vi "压力测量 - PS1.vi"(7 "CSM Name":string="PS1") -> ()   [LabVIEW 2026, in "UI-压力.lvlib"]
doc: "本范例执行串口读写操作。串口设置的参数必须匹配连接仪器或设备的参数。“VISA配置串口”VI可设置配置参数。前面板显示的控件可用于配置基本参数，如波特率、数据位和校验。VI会将VISA资源名称传递至其他VI以便执行相关操作。“VISA写入”函数将发送一个命令至串行设备，“VISA读取”函数将返回基于该命令的数据。“VISA关闭”函数可关闭该串行设备的引用。关闭引用十分重要，否则可能导致无法通过该端口进行进一步通信。"
uses:
  Supports/Device Info.ctl
  Data ColndSave/Supports/Time and Data.ctl
  <userlib>/_NEVSTOP/Communicable State Machine(CSM)/_Polymophic/CSM - Filter Duplicated Lines.vi
  3bfe9962-92bc-40b7-b1cd-a3f228b2ce0e.vi
  a504483a-bf88-4c5a-91ab-55111343aa78.vi
  83b94e39-b988-42ca-a5a6-ff8d58f134e6.vi
  5c51d1aa-81ea-4676-ad38-3af52935de4b.vi
  c16b87e5-7dba-47c4-ba33-901f1143b7c9.vi
  <userlib>/_NEVSTOP/Communicable State Machine(CSM)/_Polymophic/CSM - Replace Marks in Messages.vi
  3c314e7f-670f-419a-b1ed-a8d2dbf1e4a0.vi
  3d643602-a75e-4059-973b-e34c822a4a8c.vi
  373a0183-da7f-49bb-adc3-be145d208bff.vi
  943d190c-034f-4b86-a001-ad39c7e32d55.vi
  <userlib>/_NEVSTOP/Communicable State Machine(CSM)/AdvanceAPI/CSM - Compact Multiple States.vi
  <userlib>/_NEVSTOP/Communicable State Machine(CSM)/AdvanceAPI/CSM - Break Down Multiple States String.vi
  <userlib>/_NEVSTOP/Communicable State Machine(CSM)/_Shared/Remove Comments from Single-line.vi
  <userlib>/_NEVSTOP/Communicable State Machine(CSM)/_Shared/Split Single-line Message.vi
  <userlib>/_NEVSTOP/Communicable State Machine(CSM)/_Shared/Trim Single-line Text.vi
  <userlib>/_NEVSTOP/Communicable State Machine(CSM)/AdvanceAPI/CSM - Revert Arguments-Safe String.vi
  <userlib>/_NEVSTOP/Communicable State Machine(CSM)/AdvanceAPI/CSM - Make String Arguments Safe.vi
  5c51d1aa-81ea-4676-ad38-3af52935de4b.vi/99de0c97-112a-4c86-9094-c187659127e1.vi
  <userlib>/_NEVSTOP/Communicable State Machine(CSM)/Utility/Build Error Cluster.vi
  <vilib>/Utility/error.llb/Trim Whitespace.vi
  <vilib>/Utility/error.llb/Trim Whitespace (string).vi
  <userlib>/_NEVSTOP/Communicable State Machine(CSM)/AdvanceAPI/CSM - Keywords.vi
  <vilib>/Utility/error.llb/Trim Whitespace One-Sided.vi
  <userlib>/_NEVSTOP/Communicable State Machine(CSM)/addons/API-String-Arugments-Support/_Support/Data To API String Arguments.vi
  <userlib>/_NEVSTOP/Communicable State Machine(CSM)/addons/INI-Static-Variable-Support/_Support/instances/_CSM - Read File Logger Configuration - v1.0.vi
  <vilib>/Utility/Data Type/Get Type Information.vi
  <userlib>/_NEVSTOP/Communicable State Machine(CSM)/addons/API-String-Arugments-Support/_Support/Data To SingleElementsArray_csm.vi
  <userlib>/_NEVSTOP/Communicable State Machine(CSM)/addons/INI-Static-Variable-Support/_Support/Parse Used Session and Name.vi
  <userlib>/_NEVSTOP/Communicable State Machine(CSM)/addons/INI-Static-Variable-Support/_Support/INI-FGV(lvlibp).vi
  <userlib>/_NEVSTOP/Communicable State Machine(CSM)/addons/INI-Static-Variable-Support/_Support/Populate String with INI Variable.vi
  <userlib>/_NEVSTOP/Communicable State Machine(CSM)/addons/API-String-Arugments-Support/_Support/Convert API String Arguments to Data(variant).vi
  <userlib>/_NEVSTOP/Communicable State Machine(CSM)/addons/API-String-Arugments-Support/_Support/SingleElementsArray To Data_csm.vi
  <userlib>/_NEVSTOP/Communicable State Machine(CSM)/Communicable State Machine.lvlib
  <userlib>/_NEVSTOP/Communicable State Machine(CSM)/addons/INI-Static-Variable-Support/INI-Static-Variable-Support.lvlib
  <userlib>/_NEVSTOP/Communicable State Machine(CSM)/addons/MassData-Parameter/CSM MassData Parameter Support.lvlib
  <userlib>/_NEVSTOP/Communicable State Machine(CSM)/addons/Watchdog/CSM Watchdog.lvlib
  <userlib>/_NEVSTOP/Communicable State Machine(CSM)/addons/Logger/CSM File Logger.lvlib
  Logging/Logging.lvlib
  Acquisition/Acquisition.lvlib
  Data ColndSave/Data Collection and Save.lvlib
panel:
  in  "停止":bool
  in  "显示":enum32{"压力测量", "Status"}(tab)
  out "电压值":waveform(dbl)(graph)
  out "压力值(N)":dbl=0.5 format="%.3g"
  in  "压力设备选择":bool=TRUE
  in  "压力串口":refnum<visa-resource-name>="COM18"
  out "压力值(g)":dbl=0.5 format="%.3g"
  out "电压值":dbl=0.5 format="%.3g"
  in  "压力采集开关":bool
  out "压力(g)":waveform(dbl)(graph)
  in  "Interval(s)":dbl=0.5
  out "压力采集-错误输出":errorcluster
  out "State History":string
  in  "子程序？":bool
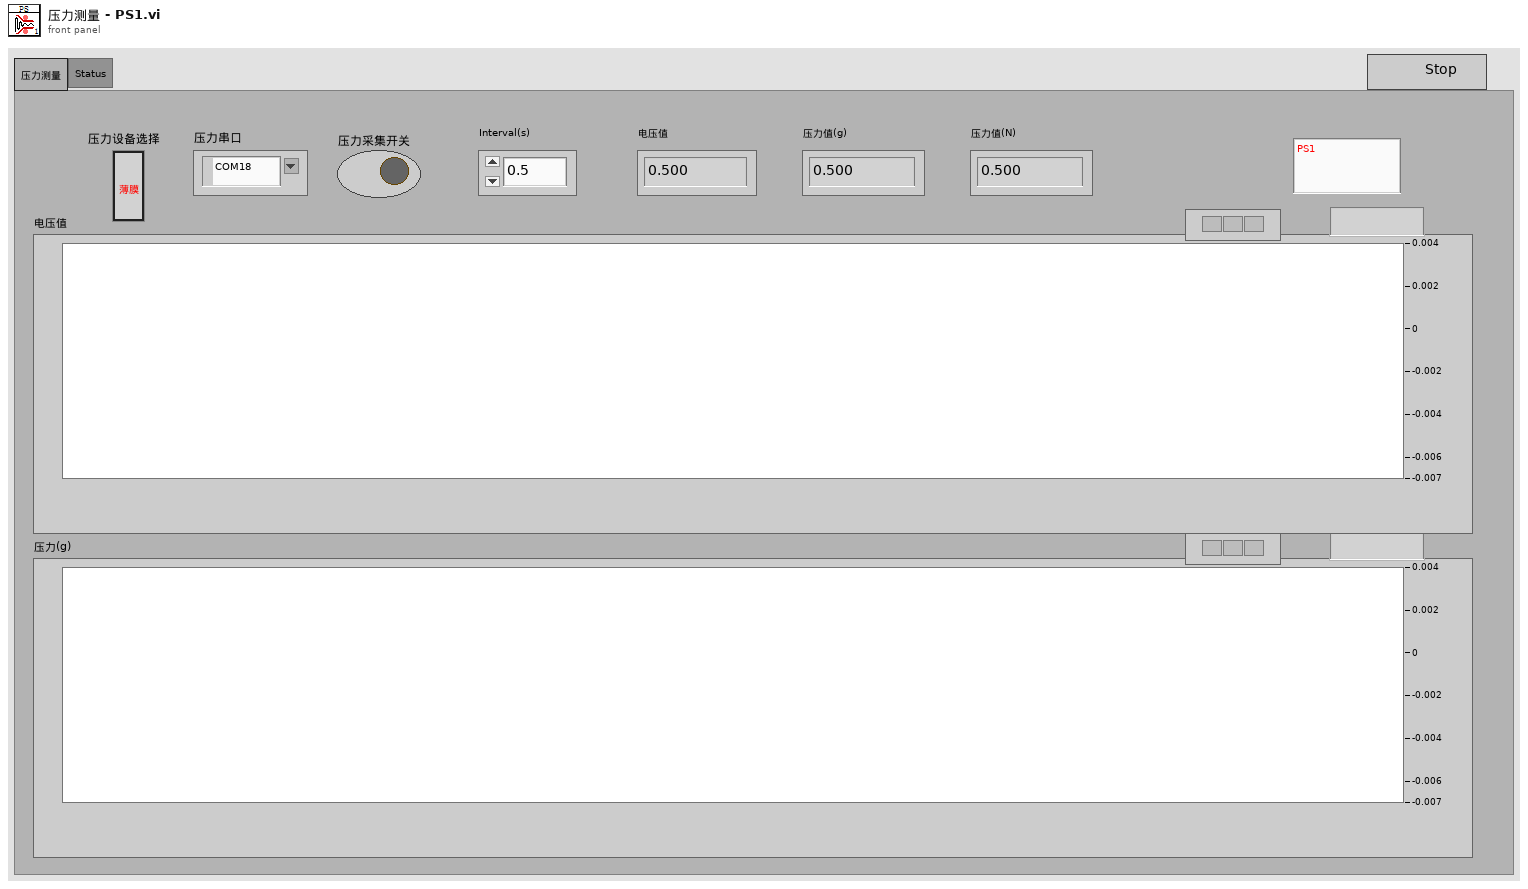
[diagram p1: front panel]
types:
  T1 = cluster{"Enable":bool, "Limit":cluster{"FileSize":i64, "FileNum":i32}, "Timestamp.Format":string, "AutoExit":bool}
  T2 = enum32{"Invalid", "Standard", "Closed", "Hidden", "Minimized", "Maximized"}
  T3 = enum32{"invalid app kind", "Development System", "Run Time System", "Student Edition", "Embedded LabVIEW", "Evaluation", "Custom"}
  T4 = typedef "Data Collection and Save.lvlib/Time and Data.ctl" = cluster{"采集时间":timestamp, "Data":dbl[]}
  T5 = typedef "Communicable State Machine.lvlib/_CSM_Response Source Message.ctl" = cluster{"‘State":string, "’Arguments":string, "’Error":errorcluster}
  T6 = cluster{"Current VI Reference":refnum<vi>, "Close Panel on Exit?":bool}
  T7 = typedef "UI-压力.lvlib/Device Info.ctl" = cluster{"USB Port":refnum<visa-resource-name>, "采集间隔(s)":dbl, "压力设备选择":bool}
  T8 = cluster{"Core":cluster{"Current VI Reference":refnum<vi>, "Close Panel on Exit?":bool}, "基本信息":T7, "Time and Data":T4, "子程序？":bool}
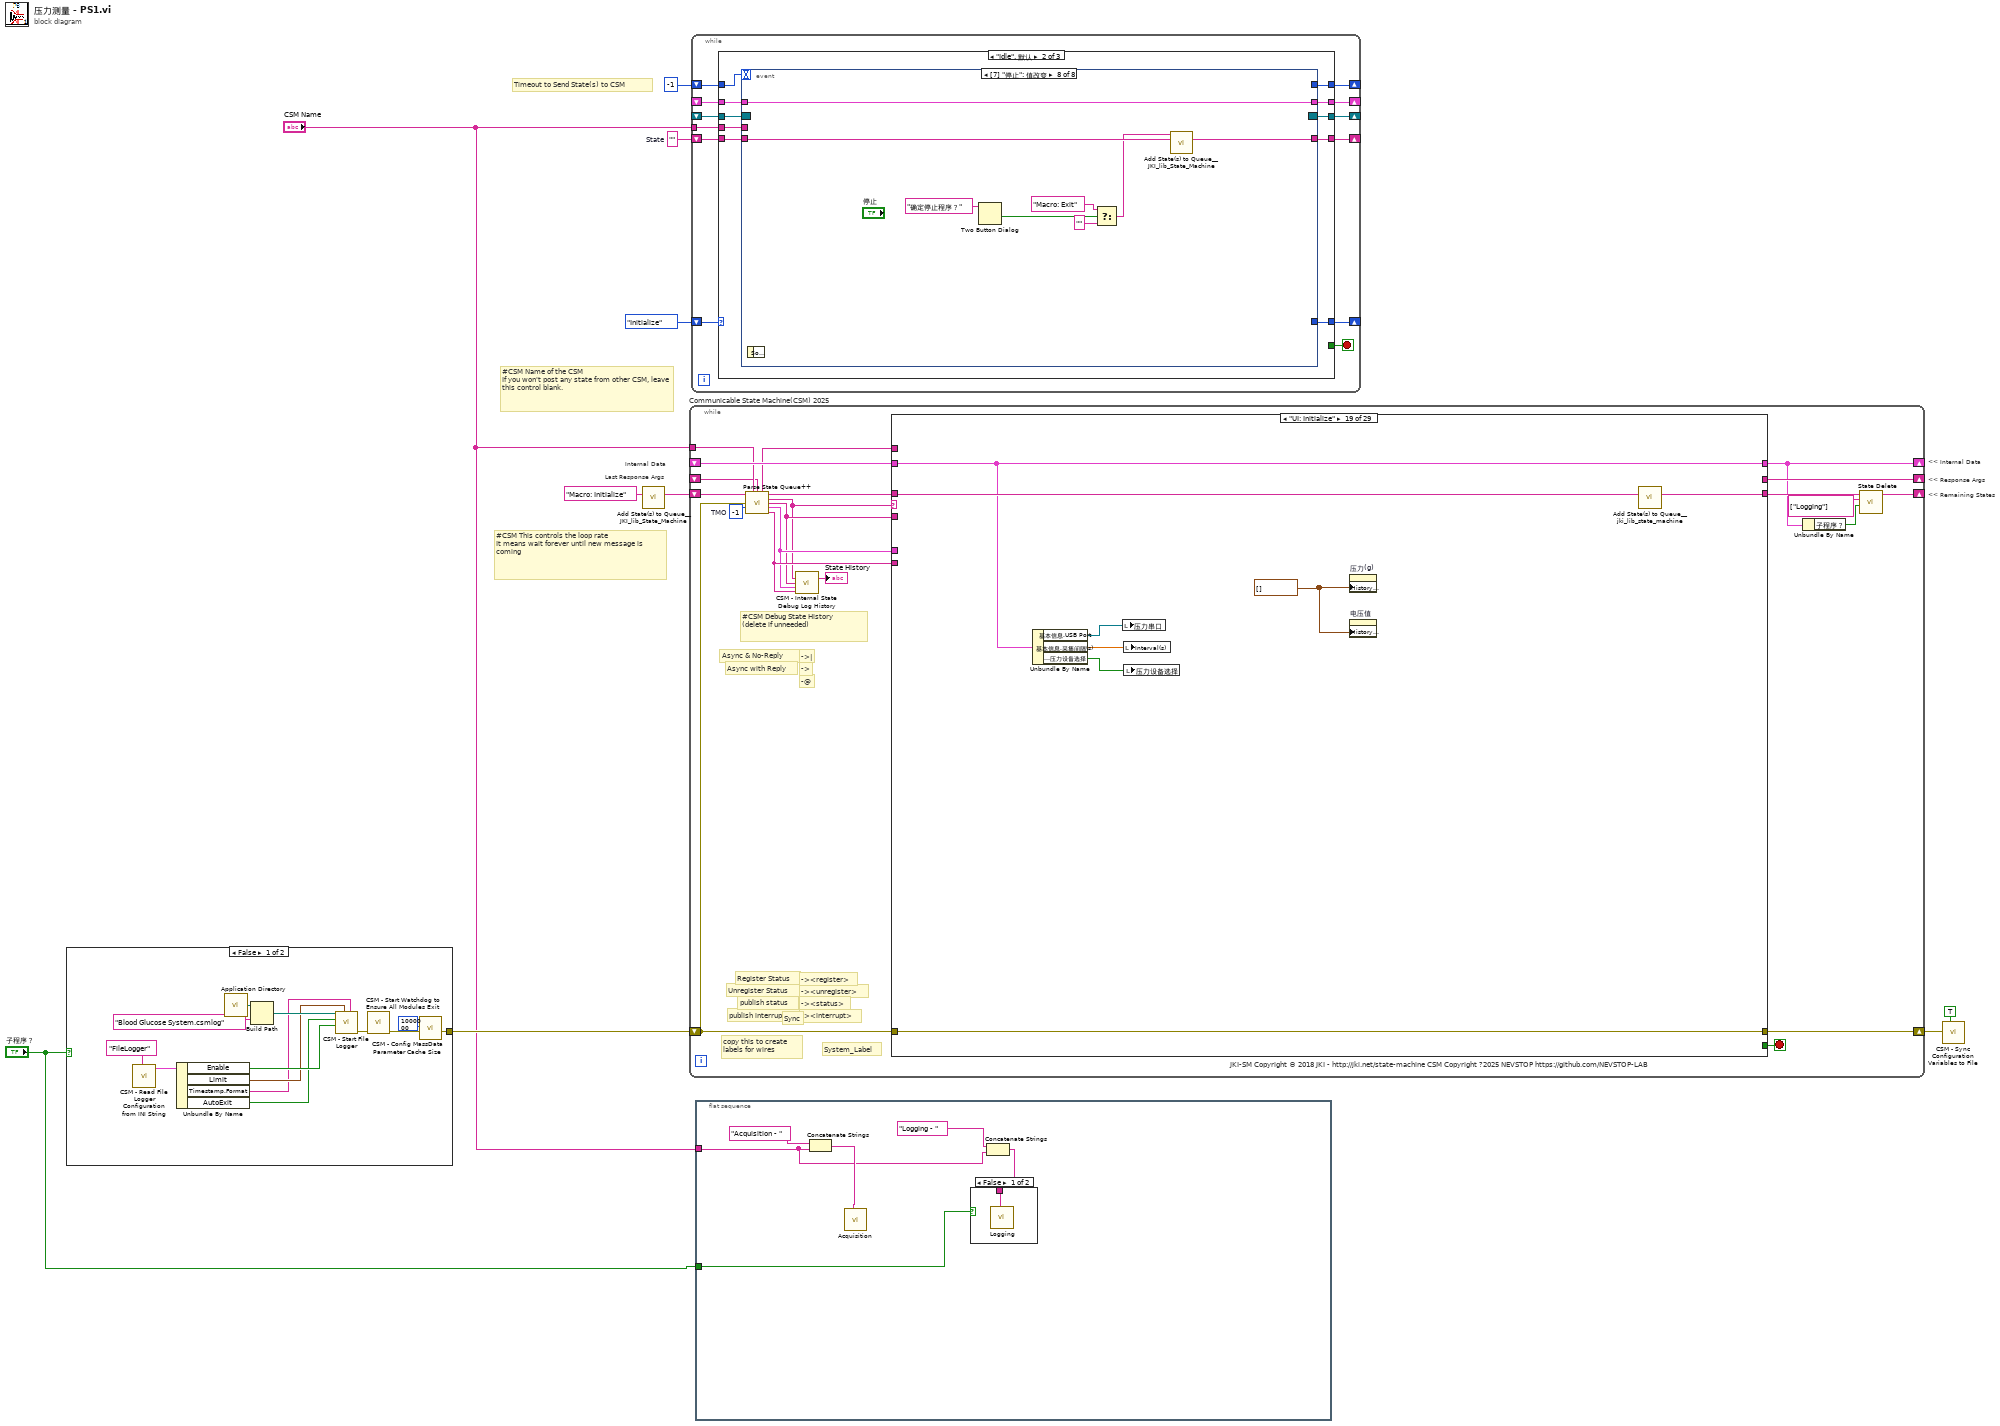
[diagram p0: block diagram]
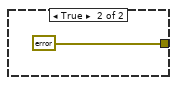
[diagram p3: hidden frame]
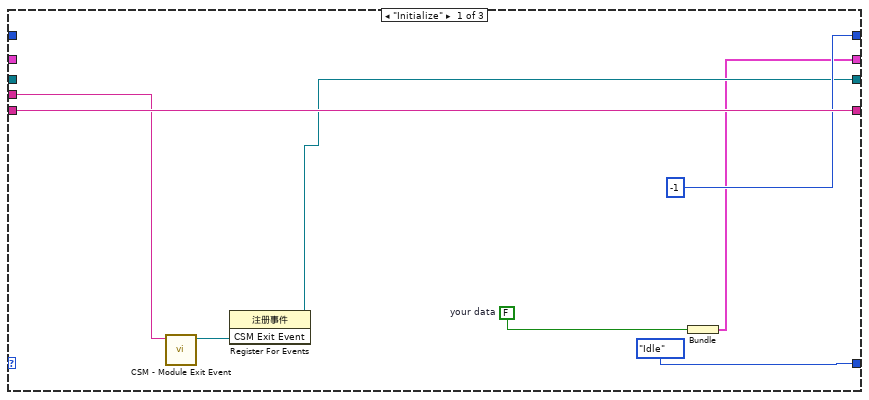
[diagram p4: hidden frame]
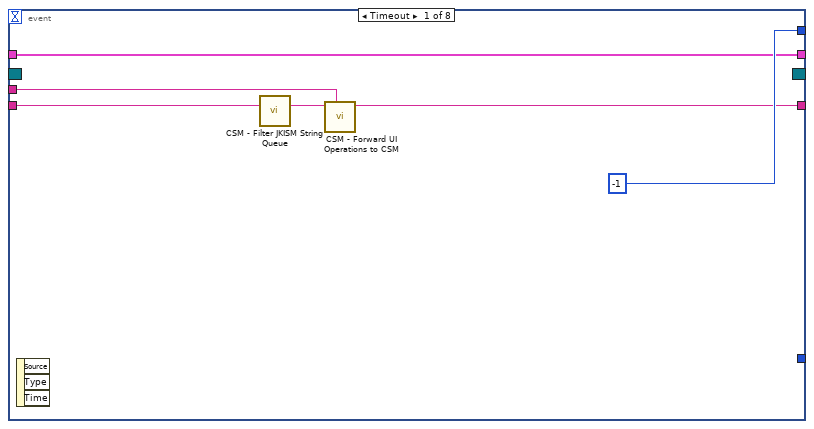
[diagram p5: hidden frame]
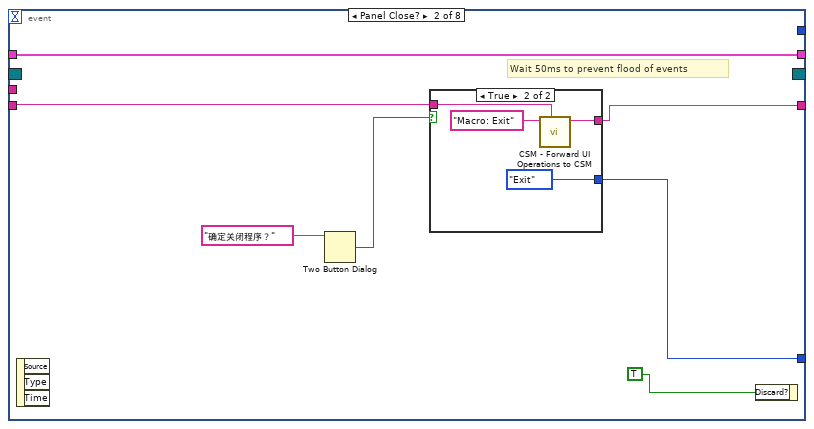
[diagram p6: hidden frame]
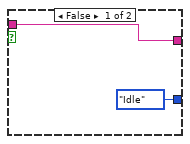
[diagram p7: hidden frame]
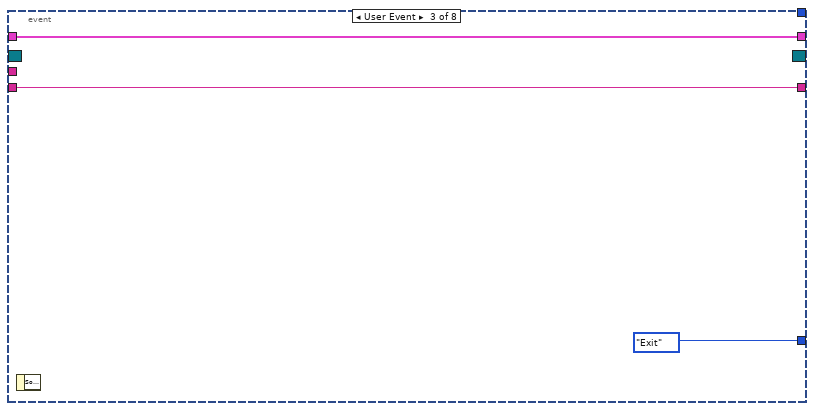
[diagram p8: hidden frame]
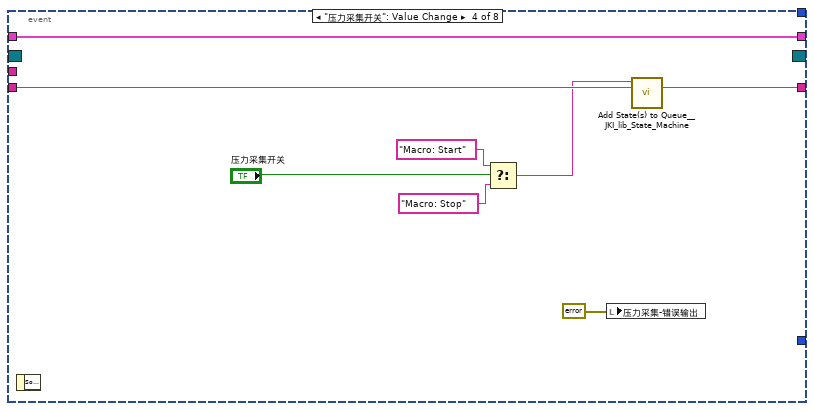
[diagram p9: hidden frame]
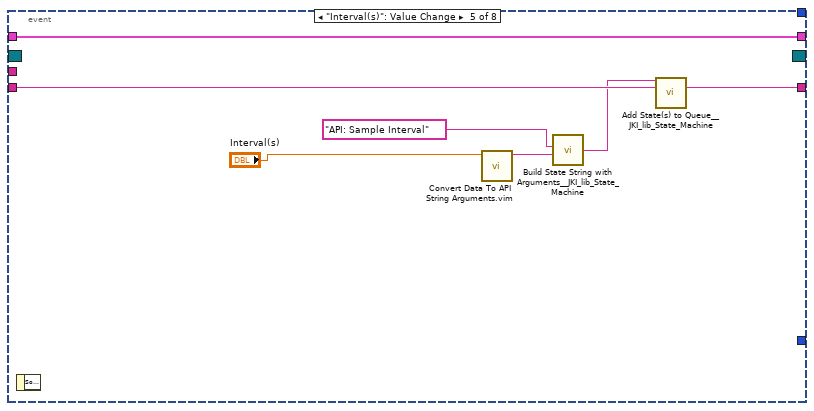
[diagram p10: hidden frame]
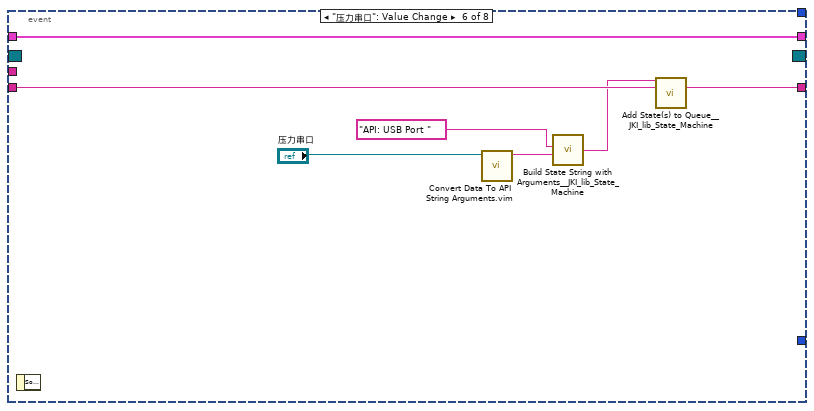
[diagram p11: hidden frame]
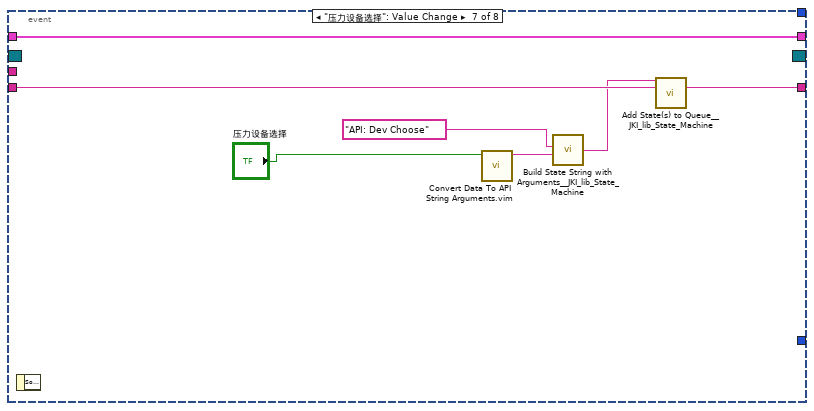
[diagram p12: hidden frame]
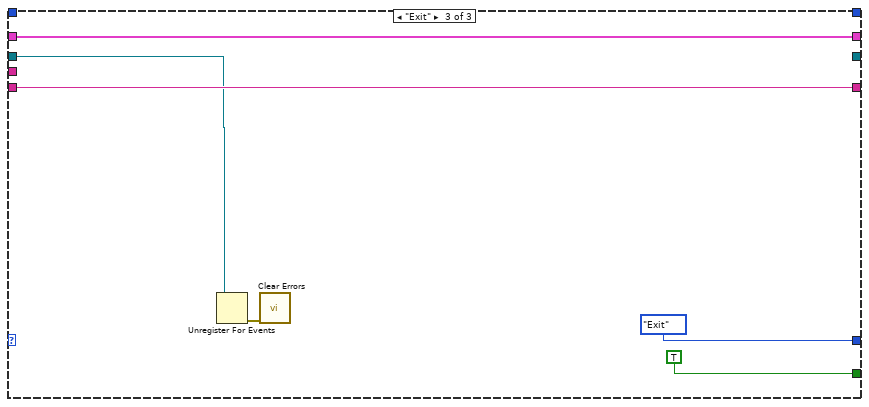
[diagram p13: hidden frame]
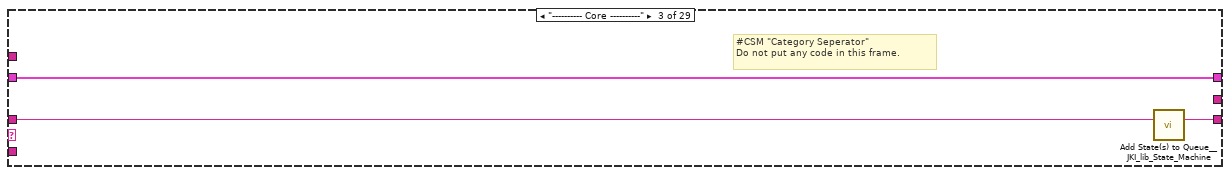
[diagram p16: hidden frame]
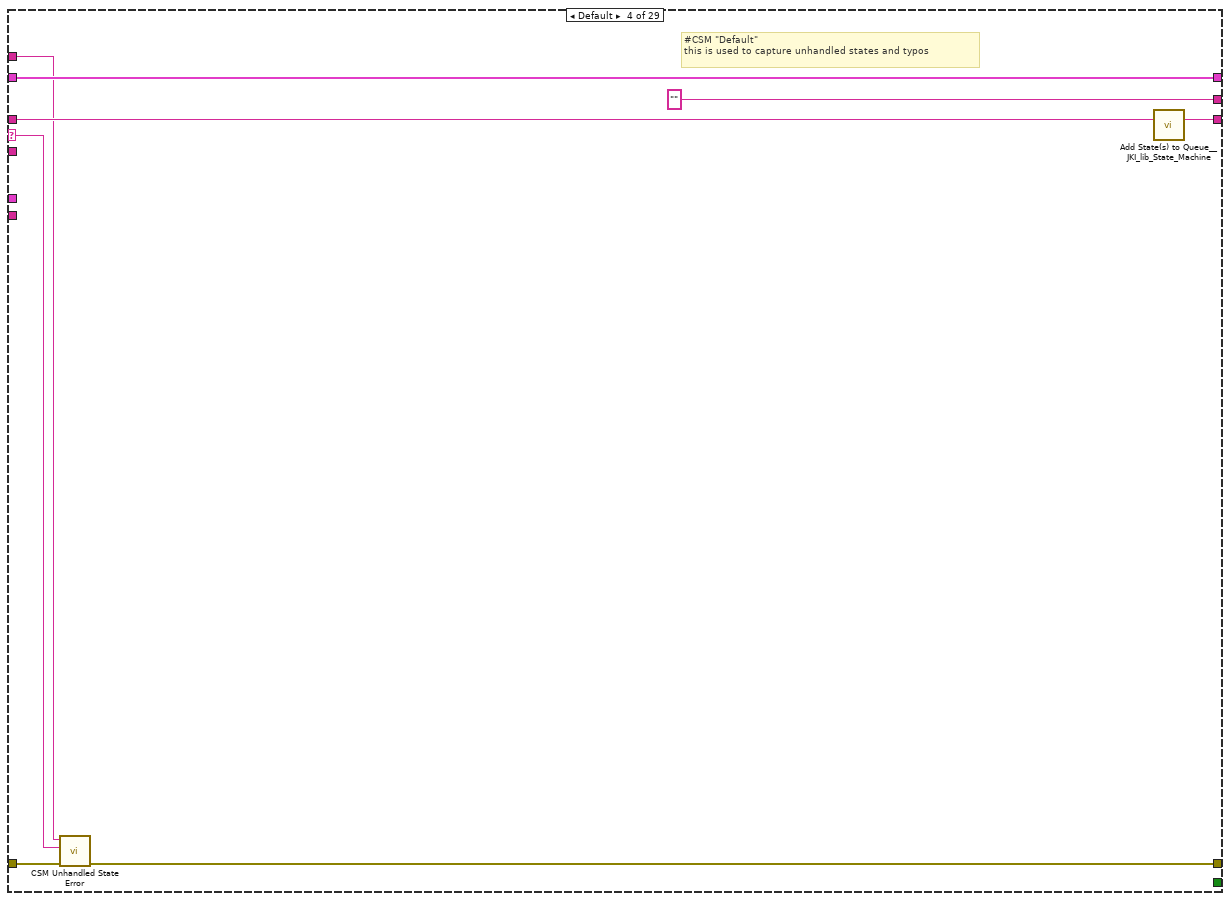
[diagram p17: hidden frame]
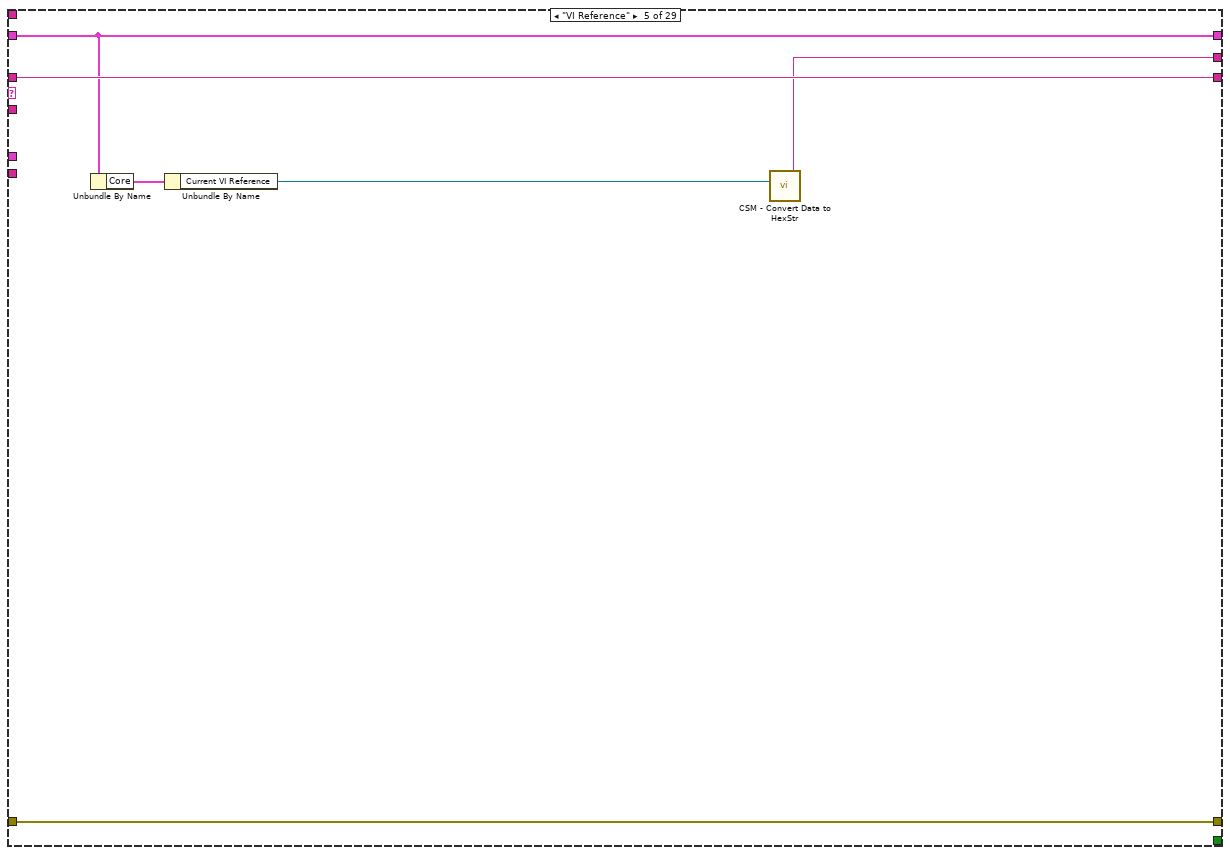
[diagram p18: hidden frame]
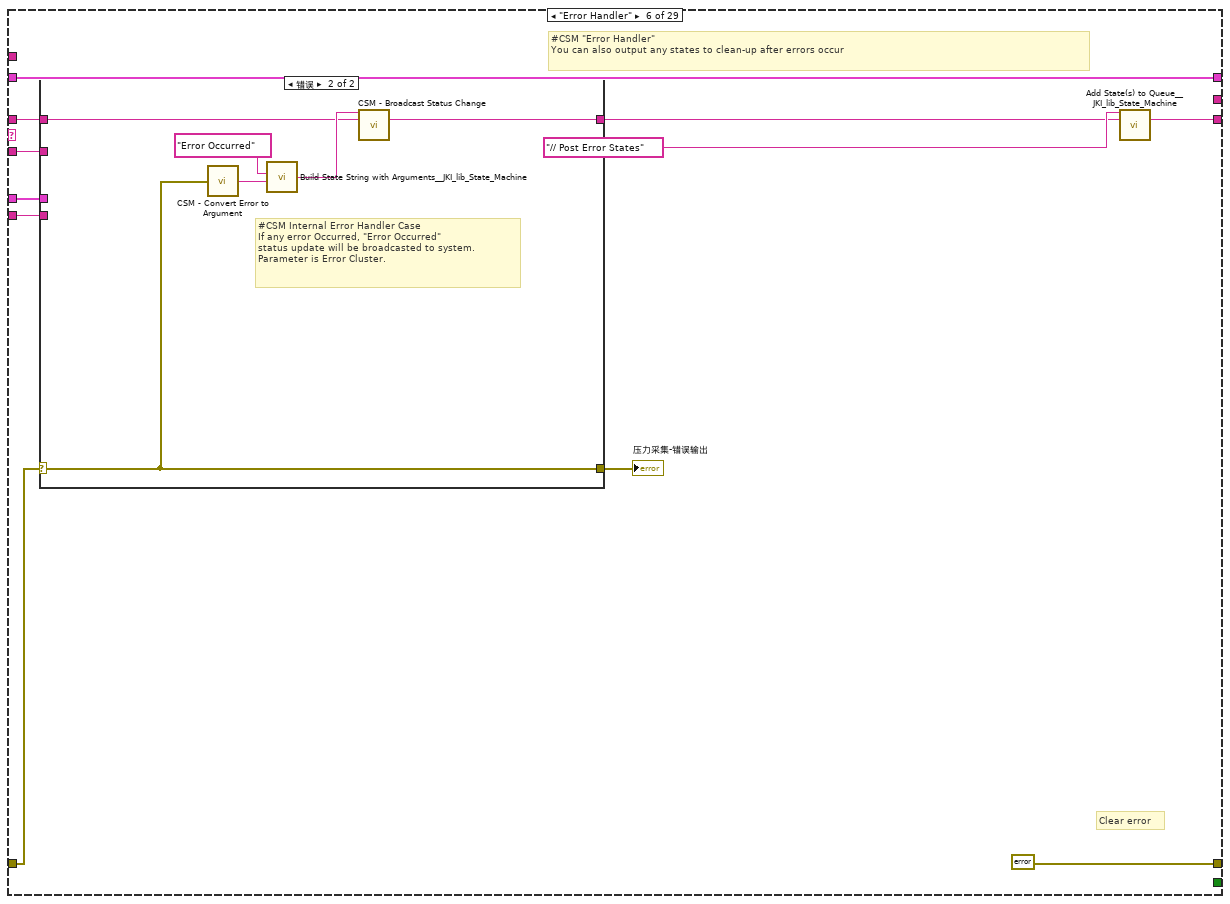
[diagram p19: hidden frame]
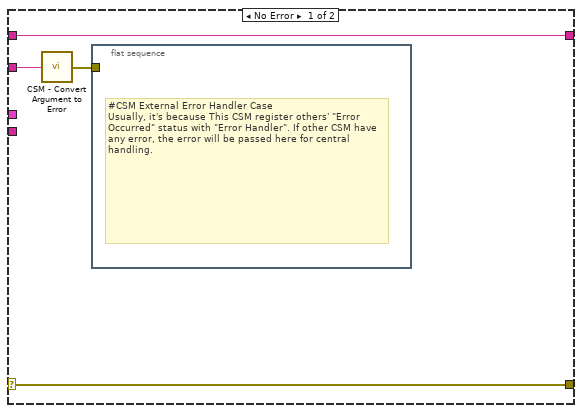
[diagram p20: hidden frame]
diagram:
  w9 = ""  # State
  # "Timeout to Send State(s) to CSM"
  # "Last Response Args"
  # "Internal Data"
  # "#CSM Name of the CSM\nIf you won't post any state from other CSM, leave this control blank."
  # "#CSM This controls the loop rate\nIt means wait forever until new message is coming"
  # "<< Internal Data"
  # "<< Response Args"
  # "<< Remaining States"
  n1 = case shown="False" "子程序？" {
    tunnel: [w21 errorcluster {"status"=FALSE, "code"=0, "source"=""} ("Error out")] -> w3
    frame False {
      n2 = call-poly <userlib>:"CSM - Read File Logger Configuration from INI String.vi"("Section Name(\"FileLogger\")"="FileLogger" ("Section Name(\"\" as Default)")) -> ("FileLogger Configuration-v1"=w15:T1)  [unwired: 7 in, 1 out]
      n3 = Unbundle By Name(w15) -> ("Enable"=w14:bool, "Limit"=w13:cluster{"FileSize":i64, "FileNum":i32}, "Timestamp.Format"=w11:string, "AutoExit"=w12:bool)
      n4 = call <vilib>:"Application Directory.vi"() -> ("Application Directory"=w20:path)
      n5 = Build Path(base path=w20, name or relative path="Blood Glucose System.csmlog") -> (appended path=w18:path)
      n6 = call <userlib>:"CSM - Start File Logger.vi"("Timestamp Format"=w11, "Log Limit"=w13, "Watchdog? (T)"=w14, "Exit When All Module Exist? (F)"=w12, "Log File Path"=w18) -> ("error out"=w17:errorcluster)  [unwired: 4 in, 2 out]
      n7 = call <userlib>:"CSM - Start Watchdog to Ensure All Modules Exit.vi"("error in (no error)"=w17) -> ("error out"=w22:errorcluster)  [unwired: 10 in]
      n8 = call <userlib>:"CSM - Config MassData Parameter Cache Size.vi"("Error in"=w22, "Size (50M)"=1000000 ("size(1M)")) -> ("Error out"=w21:errorcluster)  [unwired: 9 in]
    }
    frame True {
    }
  }
  n9 = call <vilib>:"Add State(s) to Queue__JKI_lib_State_Machine.vi"("State(s) in (\"\")"="Macro: Initialize" ("Init State(\"Macro: Initialize\")")) -> ("States Out"=w6:string)  [unwired: 14 in]
  n10 = while "Communicable State Machine(CSM) 2025" {
    shift-right: [w26] -> _
    shift-left: _ -> [w41]
    shift-right: [w43] -> w4
    shift-left: w3 -> [w31]
    shift-right: [w27] -> _
    shift-left: w6 -> [w44]
    tunnel: "CSM Name" -> [w38]
    shift-right: [w39] -> _
    shift-left: _ -> [w33]
    stop <- w42 stop-if-true
    w40 = -1  # TMO
    # "#CSM Debug State History\n(delete if unneeded)"
    # "-><interrupt>"
    # "-><status>"
    # "-><unregister>"
    # "-><register>"
    # "-@"
    # "->"
    # "->|"
    # "publish interrupt"
    # "publish status"
    # "Unregister Status"
    # "Register Status"
    # "Sync"
    # "Async with Reply"
    # "Async & No-Reply"
    # "JKI-SM Copyright © 2018 JKI - http://jki.net/state-machine CSM Copyright ?2025 NEVSTOP https://github.com/NEVSTOP-LAB"
    # "copy this to create labels for wires"
    # "System_Label"
    n11 = call <userlib>:"Parse State Queue++.vi"("State Queue"=w44, "Name (\"\" to Use UUID)"=w38, "Response Arguments"=w33, "Previous Error"=w31, "Dequeue (1 ms)"=w40) -> ("Name Used"=w32:string, "Remaining States"=w45:string, "Current State"=w34:string, "Arguments"=w35:string, "Additional Information"=w36:T5, "Source CSM"=w37:string)  [unwired: 5 in]
    n12 = call <userlib>:"CSM - Internal State Debug Log History.vi"("State"=w34, "Arguments (\"\")"=w35, ">> Response Source Message >>"=w36, "Source (\"\")"=w37) -> ("Debug Log"=→"State History":string)  [unwired: 11 in]
    n13 = case shown="\"UI: Initialize\"" w34 {
      selector: w34 -> [_ _ _ w56 _ _ _ _ _ _ _ _ _ _ _ _ _ _ _ _ _ _ _ _ _ _ _ _ _]
      tunnel: w45 -> [w46 w49 w52 w60 w65 w71 w95 w101 w107 w117 w124 w136 w140 w143 w156 w169 w178 w179 w188 w201 w206 w212 w221 w224 w235 w237 w245 w253 w260]
      tunnel: w35 -> [_ _ _ _ _ w70 w91 w98 w104 w111 _ _ _ _ _ w167 _ _ _ _ _ _ _ _ _ _ w242 w252 w259]
      tunnel: w41 -> [w47 w48 w50 w58 w64 w76 w93 w99 w105 w115 w123 w130 w138 w141 _ w160 w173 w181 w183 w193 w204 w210 w215 w228 w233 w236 w239 w250 w257]
      tunnel: [_ _ _ w53 w66 errorcluster {"status"=FALSE, "code"=0, "source"=""} ("error out") w88 w96 w102 w118 _ _ _ _ _ _ w174 w182 w190 w203 _ _ _ w229 _ _ _ _ _] -> w43
      tunnel: w31 -> [_ _ _ w54 w66 w74 w89 w97 w103 _ _ _ _ _ _ _ w175 w182 w190 w203 _ _ _ w229 _ _ _ _ _]
      tunnel: [w46 w49 w51 w59 w65 w72 w94 w100 w106 w116 w124 w135 w139 w142 w155 w170 w177 w180 w189 w202 w205 w211 w220 w225 w234 w237 w246 w254 w261] -> w28
      tunnel: [_ _ _ _ _ _ TRUE _ _ _ _ _ TRUE _ _ _ _ _ _ _ _ _ _ _ _ _ _ _ _] -> w42
      tunnel: [w47 w48 w50 w58 w64 w76 w93 w99 w105 w114 w123 w134 w138 w141 w154 w159 w173 w181 w183 w193 w204 w210 w216 w228 w233 w236 w238 w249 w256] -> w26
      tunnel: w37 -> [_ _ _ _ _ w69 _ _ _ w112 _ _ _ _ _ _ _ _ _ _ _ _ _ _ _ _ _ _ _]
      tunnel: w36 -> [_ _ _ _ _ w68 _ _ _ w113 _ _ _ _ _ _ _ _ _ _ _ _ _ _ _ _ _ _ _]
      tunnel: [_ _ _ "" w61 _ _ _ _ _ _ _ _ _ _ _ _ _ _ _ _ _ _ _ _ _ _ _ _] -> w39
      tunnel: w32 -> [_ _ _ w55 _ _ w90 _ _ _ _ _ _ _ w146 _ _ _ _ _ _ w208 _ w226 w230 _ w243 _ _]
      frame "", "Idle" {
        # "#CSM \"Idle/Event Handler\"\nexecutes when the state queue is empty"
      }
      frame "CSM Documentation" {
        # "#CSM State Syntax\n\n// Comment line, all text to the right of “//” will be ignored\n// Local Message Example\nDoSth: DoA >> Arguments\n\n// Sync Call Example\nAPI: xxxx >> Arguments -@ TargetModule\n\n// Async Call Example\nAPI: xxxx >> Arguments -> TargetModule\n\n// Async Call without Reply Example\nAPI: xxxx >> Arguments ->| TargetModule\n\n// Broadcast normal status:\nStatus >> StatusArguments  -><status>\n\n// Broadcast Interrupt status:\nInterrupt >> StatusArguments  -><interrupt>\n\n// Register Source Module's status to Handler Module\nStatus@Source Module >> Handler Module@Handler Module -><register>\n\n// Unegister Source Module's status\nStatus@Source Module >> Handler Module -><unregister>"
        # "#CSM README FIRST\n\nCommunicable State Machine(CSM) is a LabVIEW application framework that builds upon JKI State Machine(JKISM). It follows the pattern of JKISM and extends the keywords to describe message communication between modules, including concepts such as Sync-Message, Async-Message, Subscription/Unsubscription of status - essential elements for creating reusable code modules. For more information, please visit the CSM wiki: https://nevstop-lab.github.io/CSM-Wiki/\n\nFor instructions on JKI State Machine, visit: \n    http://jki.net/state-machine/\nFor information about CSM, visit: \n    https://github.com/NEVSTOP-LAB"
        # "#CSM \"Documentation\"\nCase for holding CSM Documenation"
      }
      frame "---------- Core ----------" {
        # "#CSM \"Category Seperator\"\nDo not put any code in this frame."
        n14 = call <vilib>:"Add State(s) to Queue__JKI_lib_State_Machine.vi"("State(s) in (\"\")"=w52) -> ("States Out"=w51:string)  [unwired: 14 in]
      }
      frame Default {
        # "#CSM \"Default\"\nthis is used to capture unhandled states and typos"
        n15 = call <userlib>:"CSM Unhandled State Error.vi"("error in (no error)"=w54, "Undefined State"=w56, "CSM Name"=w55) -> ("error out"=w53:errorcluster)  [unwired: 8 in]
        n16 = call <vilib>:"Add State(s) to Queue__JKI_lib_State_Machine.vi"("State(s) in (\"\")"=w60) -> ("States Out"=w59:string)  [unwired: 14 in]
      }
      frame "VI Reference" {
        n17 = Unbundle By Name(w64) -> ("Core"=w63:T6)
        n18 = Unbundle By Name(w63) -> ("Current VI Reference"=w62:refnum<vi>)
        n19 = call <userlib>:"CSM - Convert Data to HexStr.vi"("Variant"=w62) -> ("HEX String (0-9,A-F)"=w61:string)  [unwired: 8 in]
      }
      frame "Error Handler" {
        # "#CSM \"Error Handler\"\nYou can also output any states to clean-up after errors occur"
        # "Clear error"
        n20 = case shown="错误" w74 {
          selector: w74 -> [w78 w82]
          tunnel: [w81 w84] -> w73
          tunnel: w71 -> [w81 w83]
          tunnel: w70 -> [w80 _]
          tunnel: w69 -> [_ _]
          tunnel: w68 -> [_ _]
          tunnel: [w78 w82] -> w67
          frame No Error {
            n21 = call <userlib>:"CSM - Convert Argument to Error.vi"("Argument"=w80) -> ("Error"=w79:errorcluster)  [unwired: 4 in]
            n22 = flat-sequence {
              tunnel: w79 -> [_]
              frame #0 {
                # "#CSM External Error Handler Case\nUsually, it's because This CSM register others' \"Error Occurred\" status with \"Error Handler\". If other CSM have any error, the error will be passed here for central handling."
              }
            }
          }
          frame Error {
            # "#CSM Internal Error Handler Case \nIf any error Occurred, \"Error Occurred\" \nstatus update will be broadcasted to system.\nParameter is Error Cluster."
            n23 = call <userlib>:"CSM - Convert Error to Argument.vi"("Error"=w82) -> ("Argument"=w86:string)  [unwired: 4 in]
            n24 = call <vilib>:"Build State String with Arguments__JKI_lib_State_Machine.vi"("Arguments (\"\")"=w86, "State"="Error Occurred" ("Status with Arguments")) -> ("State with Arguments"=w85:string)  [unwired: 4 in]
            n25 = call <userlib>:"CSM - Broadcast Status Change.vi"("Status With Arguments"=w85, "State Queue"=w83) -> ("Remaining States"=w84:string)  [unwired: 13 in]
          }
        }
        "压力采集-错误输出" <- w67
        n26 = call <vilib>:"Add State(s) to Queue__JKI_lib_State_Machine.vi"("State(s) in Front (\"\")"="// Post Error States", "State(s) in (\"\")"=w73) -> ("States Out"=w72:string)  [unwired: 13 in]
      }
      frame "Critical Error" {
        # "#CSM \"Critical Error\"\nWhen any un-recoverable error occurs, CSM goes into this case."
        # "#CSM Stop in Critical Error\nWhen Critical Error occurs, Stop the loop immediately. Do NOT change this unless you fully understand the impact."
        n27 = call <userlib>:"CSM Critical Error.vi"("error in (no error)"=w89, "Arugments (As Reason)"=w91, "CSM Name"=w90) -> ("error out"=w88:errorcluster)  [unwired: 8 in]
        n28 = call <vilib>:"Add State(s) to Queue__JKI_lib_State_Machine.vi"("State(s) in (\"\")"=w95) -> ("States Out"=w94:string)  [unwired: 14 in]
      }
      frame "Target Timeout Error" {
        # "#CSM \"Target Timeout Error\"\nWhen This CSM could not get the sync-call response in time, This CSM goes into this case."
        n29 = call <userlib>:"CSM Target Timeout Error.vi"("error in (no error)"=w97, "Arguments (As CSM Name)"=w98) -> ("error out"=w96:errorcluster)  [unwired: 9 in]
        n30 = call <vilib>:"Add State(s) to Queue__JKI_lib_State_Machine.vi"("State(s) in (\"\")"=w101) -> ("States Out"=w100:string)  [unwired: 14 in]
      }
      frame "Target Error" {
        # "#CSM \"Target Error\"\nWhen This CSM try to communicate with an un-existed CSM, This CSM goes into this case."
        n31 = call <userlib>:"CSM Target Error.vi"("error in (no error)"=w103, "Arguments (As CSM Name)"=w104) -> ("error out"=w102:errorcluster)  [unwired: 9 in]
        n32 = call <vilib>:"Add State(s) to Queue__JKI_lib_State_Machine.vi"("State(s) in (\"\")"=w107) -> ("States Out"=w106:string)  [unwired: 14 in]
      }
      frame "Async Response", "Response" {
        n33 = Unbundle(w113) -> ("‘State"=w110:string, "’Arguments"=w109:string, "’Error"=w108:errorcluster)
        n34 = case shown="默认" w110 {
          tunnel: [w119] -> w116
          tunnel: w117 -> [w120]
          tunnel: [w122] -> w114
          tunnel: w115 -> [w122]
          tunnel: [w121] -> w118
          tunnel: w108 -> [w121]
          tunnel: w112 -> [_]
          tunnel: w111 -> [_]
          tunnel: w109 -> [_]
          frame 默认 {
            # "#CSM \"Async Response\"\nHandle Async-call Response (\"Async Response\" for ->)"
            # "#CSM \"Response\"\nHandle Sync-call Response (\"Response\" for -@)"
            # "#CSM Response Comments\nAfter Message is executed, CSM goes to this state for receive the response.\n    For Async Message(->), \"Async Response\" is used. This CSM will goes to \"Async Message Posted\" immediately and receive the \"Async Response\" after the callee finishes the message.\n    For Sync Message(@),  This CSM will wait until the message is done and immediately goes to \"Response\""
            n35 = call <vilib>:"Add State(s) to Queue__JKI_lib_State_Machine.vi"("State(s) in (\"\")"=w120) -> ("States Out"=w119:string)  [unwired: 14 in]
          }
        }
      }
      frame "Async Message Posted" {
        # "#CSM \"Async Message Posted\"\nAfter Async Message is posted (-> or ->| ), CSM goes to this state for post-action.\nYou can use Argument - State to tell which Async Message is called."
      }
      frame "Initialize Core Data" {
        # "#CSM \"Initialize Core Data\"\nThis is used to determine panel behavior on exit"
        # "originally closed?"
        # "exe?"
        # "If panel starts closed or is an EXE, then close it when we exit"
        n36 = property class="VI"() -> ("FP.State"=w127:T2)  [unwired: 2 in, 2 out]
        n37 = property class="App"() -> ("App.Kind"=w133:T3)  [unwired: 2 in, 2 out]
        n38 = control-ref of="Current VI Reference"() -> (w128:refnum<vi>)
        n39 = Equal?(x=w127, y=T2."Closed" ("Front Panel Window:State")) -> (x = y?=w125:bool)
        n40 = Equal?(x=w133, y=T3."Run Time System" ("Application:Kind")) -> (x = y?=w131:bool)
        n41 = Or(x=w125, y=w131) -> (x .or. y?=w129:bool)
        n42 = Bundle By Name(cluster=w130, "Core.Current VI Reference"=w128, "Core.Close Panel on Exit?"=w129) -> (w134:T8)
        n43 = call <vilib>:"Add State(s) to Queue__JKI_lib_State_Machine.vi"("State(s) in (\"\")"=w136) -> ("States Out"=w135:string)  [unwired: 14 in]
      }
      frame "Exit" {
        # "#CSM \"Exit\"\nCase for exiting the loop. No errors that occur here will be handled."
        n44 = call <vilib>:"Add State(s) to Queue__JKI_lib_State_Machine.vi"("State(s) in (\"\")"=w140) -> ("States Out"=w139:string)  [unwired: 14 in]
      }
      frame "---------- Data ----------" {
        # "#CSM \"Category Seperator\"\nDo not put any code in this frame."
        n45 = call <vilib>:"Add State(s) to Queue__JKI_lib_State_Machine.vi"("State(s) in (\"\")"=w143) -> ("States Out"=w142:string)  [unwired: 14 in]
      }
      frame "Data: Initialize" {
        w147 = T7 {"USB Port"="COM1", "采集间隔(s)"=0.5, "压力设备选择"=TRUE} ("基本信息")
        w153 = T6 {"Current VI Reference"=refnum, "Close Panel on Exit?"=FALSE}  # Core
        # "#CSM \"Data: Initialize\"\nInitialize the shift-register data, here.\n(data names are defined by what you wire into the bundle function)"
        # "#CSM do not delete - used by framework"
        # "#CSM Data names and types of shift register data are defined by this bundle."
        n46 = local read "子程序？"() -> (w150:bool)
        n47 = call "CSM - Read Cluster Elements From Session.vim"("Section Name (\"\" as Default)"=w146, "Cluster"=w147) -> ("Cluster out"=w148:T7)  [unwired: 6 in, 1 out]
        n48 = Select(t=w148, s=TRUE, f=w147) -> (s? t:f=w145:T7)
        n49 = local write "压力采集开关"(FALSE ("压力采集开关")) -> ()
        n50 = local write "压力采集-错误输出"(errorcluster {"status"=FALSE, "code"=0, "source"=""} ("压力采集-错误输出")) -> ()
        n51 = Bundle("Core"=w153, "基本信息"=w145, "Time and Data"=T4 {"采集时间"=timestamp(0 s since 1904-01-01), "Data"=[0.0, 0.0]}, "子程序？"=w150) -> (w154:T8)  [unwired: 1 in]
        n52 = call <vilib>:"Add State(s) to Queue__JKI_lib_State_Machine.vi"("State(s) in (\"\")"=w156) -> ("States Out"=w155:string)  [unwired: 14 in]
      }
      frame "Data: Update Indicators" {
        n53 = call "Convert API String Arguments to Data.vim"("Reference Type"=T4 {"采集时间"=timestamp(0 s since 1904-01-01), "Data"=[]} ("Time and Data"), "API String"=w167) -> ("Data"=w165:T4)  [unwired: 6 in, 1 out]
        n54 = Unbundle By Name(w165) -> ("采集时间"=w158:timestamp, "Data"=w157:dbl[])
        n55 = Index Array(array=w157) -> (element #1=→"电压值":dbl, element #2=w162:dbl)  [unwired: 2 in]
        "压力值(g)" <- w162
        n56 = Divide(x=w162, y=100.0) -> (x/y=→"压力值(N)":dbl)
        n57 = in-place {
          in-place-border: w158 -> [w172]
          in-place-border: w157 -> [w171]
          n58 = in-place-cluster #1(w160) -> ()  [unwired: 2 out]
          n59 = in-place-cluster #1("Time and Data.采集时间"=w172, "Time and Data.Data"=w171) -> (w159:T8)
        }
        n60 = call <vilib>:"Add State(s) to Queue__jki_lib_state_machine.vi"("State(s) in Front (\"\")"="UI: Update Graph" ("State(s) in Front (\"\")"), "State(s) in (\"\")"=w169) -> ("States Out"=w170:string)  [unwired: 13 in]
      }
      frame "Data: Cleanup" {
        # "#CSM \"Data: Cleanup\"\nCleanup any data and references, here.\n(this is called automatically, by the Macro: Exit)"
        n61 = Unbundle By Name(w173) -> ("Core.Current VI Reference"=w176:refnum<vi>)
        n62 = Close Reference(reference=w176, error in (no error)=w175) -> (error out=w174:errorcluster)
        n63 = call <vilib>:"Add State(s) to Queue__JKI_lib_State_Machine.vi"("State(s) in (\"\")"=w178) -> ("States Out"=w177:string)  [unwired: 14 in]
      }
      frame "---------- UI ----------" {
        n64 = call <vilib>:"Add State(s) to Queue__jki_lib_state_machine.vi"("State(s) in (\"\")"=w179) -> ("States Out"=w180:string)  [unwired: 14 in]
      }
      frame "UI: Initialize" {
        w187 = waveform(dbl)[] [] ("历史数据")
        n65 = Unbundle By Name(w183) -> ("基本信息.USB Port"=w184:refnum<visa-resource-name>, "基本信息.采集间隔(s)"=w186:dbl, "基本信息.压力设备选择"=w185:bool)
        n66 = local write "压力串口"(w184) -> ()
        n67 = local write "Interval(s)"(w186) -> ()
        n68 = local write "压力设备选择"(w185) -> ()
        n69 = property on="压力(g)" class="WFChart (严格)"("History Data"=w187) -> ()  [unwired: 2 in, 2 out]
        n70 = property on="电压值" class="WFChart (严格)"("History Data"=w187) -> ()  [unwired: 2 in, 2 out]
        n71 = call <vilib>:"Add State(s) to Queue__jki_lib_state_machine.vi"("State(s) in (\"\")"=w188) -> ("States Out"=w189:string)  [unwired: 14 in]
      }
      frame "UI: Update Graph" {
        n72 = Unbundle By Name(w193) -> ("Time and Data.Data"=w199:dbl[], "Time and Data.采集时间"=w197:timestamp, "基本信息.采集间隔(s)"=w196:dbl)
        n73 = Index Array(array=w199) -> (element #1=w192:dbl, element #2=w191:dbl)  [unwired: 2 in]
        n74 = Build Array(w191) -> (w200:dbl[])
        n75 = Build Array(w192) -> (w198:dbl[])
        n76 = Bundle By Name("Y"=w200, "t0"=w197, "dt"=w196) -> (→"压力(g)":waveform(dbl))  [unwired: 1 in]
        n77 = Bundle By Name("Y"=w198, "t0"=w197, "dt"=w196) -> (→"电压值":waveform(dbl))  [unwired: 1 in]
        n78 = call <vilib>:"Add State(s) to Queue__jki_lib_state_machine.vi"("State(s) in (\"\")"=w201) -> ("States Out"=w202:string)  [unwired: 14 in]
      }
      frame "---------- Macro ----------" {
        # "#CSM \"Category Seperator\"\nDo not put any code in this frame."
        n79 = call <vilib>:"Add State(s) to Queue__JKI_lib_State_Machine.vi"("State(s) in (\"\")"=w206) -> ("States Out"=w205:string)  [unwired: 14 in]
      }
      frame "Macro: Initialize" {
        w209 = "Data: Initialize\nInitialize Core Data\nUI: Initialize\n\n//Permanent registrations\nAcquired Data@Acquisition - <1> >> Data: Update Indicators -><register>\nAcquired Data@Acquisition - <1> >> API: Log@Logging - <1> -><register>\n\n//Error registrations\nError Occurred@Acquisition - <1> >> Error Handler -><register>\nError Occurred@Logging - <1> >> Error Handler -><register>\n\n//Dynamic registrations\n// 订阅/取消订阅\n//Status@SourceModule >> API@TargetModule -><register as interrupt>\n//UrgentEvent @SourceModule >> API@TargetModule -><register as status>\n\n\n\n//Launch Acquisition Module\n"  # Data: Initialize Initialize Core Data UI: Initialize  //Permanent registrations Acquired Data@Acquisition - <1> >> Data: Update Indicators -><register> Acquired Data@Acquisition - <1> >> API: Log@Logging - <1> -><register>  //Error registrations Error Occurred@Acquisition - <1> >> Error Handler -><register> Error Occurred@Logging - <1> >> Error Handler -><register>  //Dynamic registrations // 订阅/取消订阅 //Status@SourceModule >> API@TargetModule -><register as interrupt> //UrgentEvent @SourceModule >> API@TargetModule -><register as status>    //Launch Acquisition Module
        n80 = call-poly <userlib>:"Build Message with Arguments++.vi"("States With Replace Token"=w209, "<1>"=w208) -> ("States"=w207:string)  [unwired: 13 in]
        n81 = call <vilib>:"Add State(s) to Queue__JKI_lib_State_Machine.vi"("State(s) in Front (\"\")"=w207, "State(s) in (\"\")"=w212) -> ("States Out"=w211:string)  [unwired: 13 in]
      }
      frame "Macro: Start" {
        # "#CSM \"Macro: Initialize\"\nInitialization Macro (This is called once, when the VI starts)"
        n82 = Unbundle By Name(w215) -> ("基本信息"=w214:T7)
        n83 = local write "压力采集开关"(TRUE ("压力采集开关")) -> ()
        n84 = call "Convert Data To API String Arguments.vim"("Data"=w214) -> ("API String"=w218:string)  [unwired: 7 in, 1 out]
        n85 = call-poly <userlib>:"Build Message with Arguments++.vi"("States With Replace Token"="API: Start >> <param> -@ Acquisition - <1>\nAPI: Start  -@ Logging - <1>" ("State"), "<param>"=w218) -> ("States"=w217:string)  [unwired: 13 in]
        n86 = call <vilib>:"Add State(s) to Queue__JKI_lib_State_Machine.vi"("State(s) in Front (\"\")"=w217, "State(s) in (\"\")"=w221) -> ("States Out"=w220:string)  [unwired: 13 in]
        n87 = Bundle By Name(cluster=w215, "基本信息"=w214) -> (w216:T8)
      }
      frame "Macro: Stop" {
        n88 = local write "压力采集开关"(FALSE ("压力采集开关")) -> ()
        n89 = call-poly <userlib>:"Build Message with Arguments++.vi"("States With Replace Token"="//Send Message to Other CSM Modules\nAPI: Stop -@ Acquisition - <1>\nAPI: Stop -@ Logging - <1>", "<1>"=w226) -> ("States"=w223:string)  [unwired: 13 in]
        n90 = call <vilib>:"Add State(s) to Queue__jki_lib_state_machine.vi"("State(s) in Front (\"\")"=w223, "State(s) in (\"\")"=w224) -> ("States Out"=w225:string)  [unwired: 13 in]
      }
      frame "Macro: Exit" {
        w232 = "//Exit\nMacro: Exit-@Acquisition - <1>\nMacro: Exit-@Logging - <1>\n\n//Permanent unregistrations\nAcquired Data@Acquisition - <1> >> Data: Update Indicators -><unregister>\nAcquired Data@Acquisition - <1> >> API: Log@Logging - <1> -><unregister>\n\n//Permanent unregistrations\nError Occurred@Acquisition - <1> >> Error Handler -><unregister>\nError Occurred@Logging - <1> >> Error Handler -><unregister>\n\nData: Cleanup\nExit"  # //Exit Macro: Exit-@Acquisition - <1> Macro: Exit-@Logging - <1>  //Permanent unregistrations Acquired Data@Acquisition - <1> >> Data: Update Indicators -><unregister> Acquired Data@Acquisition - <1> >> API: Log@Logging - <1> -><unregister>  //Permanent unregistrations Error Occurred@Acquisition - <1> >> Error Handler -><unregister> Error Occurred@Logging - <1> >> Error Handler -><unregister>  Data: Cleanup Exit
        # "#CSM \"Macro: Exit\"\nExit Macro (This is called once, when the VI exits)"
        n91 = call-poly <userlib>:"Build Message with Arguments++.vi"("States With Replace Token"=w232, "<1>"=w230) -> ("States"=w231:string)  [unwired: 13 in]
        n92 = call <vilib>:"Add State(s) to Queue__JKI_lib_State_Machine.vi"("State(s) in Front (\"\")"=w231, "State(s) in (\"\")"=w235) -> ("States Out"=w234:string)  [unwired: 13 in]
      }
      frame "---------- API ----------" {
        # "#CSM \"Category Seperator\"\nDo not put any code in this frame."
      }
      frame "API: Sample Interval" {
        # "#CSM API Example\nCopy/Rename this case for your own API"
        n93 = call "Convert API String Arguments to Data.vim"("Reference Type"=0.5 ("Interval(s)"), "API String"=w242) -> ("Data"=w240:dbl)  [unwired: 6 in, 1 out]
        n94 = call-poly <userlib>:"Build Message with Arguments++.vi"("States With Replace Token"="API: Sample Interval >> <param> ->| Acquisition - <1>" ("State"), "<param>"=w242, "<1>"=w243) -> ("States"=w244:string)  [unwired: 12 in]
        n95 = call <vilib>:"Add State(s) to Queue__jki_lib_state_machine.vi"("State(s) in Front (\"\")"=w244, "State(s) in (\"\")"=w245) -> ("States Out"=w246:string)  [unwired: 13 in]
        n96 = Bundle By Name(cluster=w239, "基本信息.采集间隔(s)"=w240) -> (w238:T8)
      }
      frame "API: USB Port" {
        # "#CSM API Example\nCopy/Rename this case for your own API"
        n97 = call "Convert API String Arguments to Data.vim"("Reference Type"=refnum<visa-resource-name> "COM18" ("压力串口"), "API String"=w252) -> ("Data"=w251:refnum<visa-resource-name>)  [unwired: 6 in, 1 out]
        n98 = call <vilib>:"Add State(s) to Queue__jki_lib_state_machine.vi"("State(s) in (\"\")"=w253) -> ("States Out"=w254:string)  [unwired: 14 in]
        n99 = Bundle By Name(cluster=w250, "基本信息.USB Port"=w251) -> (w249:T8)
      }
      frame "API: Dev Choose" {
        # "#CSM API Example\nCopy/Rename this case for your own API"
        n100 = call "Convert API String Arguments to Data.vim"("Reference Type"=TRUE ("压力设备选择"), "API String"=w259) -> ("Data"=w258:bool)  [unwired: 6 in, 1 out]
        n101 = call <vilib>:"Add State(s) to Queue__jki_lib_state_machine.vi"("State(s) in (\"\")"=w260) -> ("States Out"=w261:string)  [unwired: 14 in]
        n102 = Bundle By Name(cluster=w257, "基本信息.压力设备选择"=w258) -> (w256:T8)
      }
    }
    n103 = Unbundle By Name(w26) -> ("子程序？"=w25:bool)
    n104 = call "State Delete.vi"("Delete?(F)"=w25, "CSM name to delete"=string[] ["Logging"], "State In"=w28) -> ("State Out"=w27:string)  [unwired: 8 in]
  }
  n105 = while {
    shift-right: [w272] -> _
    shift-left: enum16{"Idle", "Initialize", "Exit"}."Initialize" -> [w273]
    tunnel: "CSM Name" -> [w270]
    shift-right: [w268] -> _
    shift-left: w9 -> [w269]
    shift-right: [w266] -> _
    shift-left: -1 -> [w267]
    shift-right: [w265] -> _
    shift-left: _ -> [w264]
    shift-right: [w263] -> _
    shift-left: _ -> [w262]
    stop <- w271 stop-if-true
    n106 = case shown="\"Idle\", 默认" w273 {
      tunnel: [enum16{"Idle", "Initialize", "Exit"}."Idle" w291 enum16{"Idle", "Initialize", "Exit"}."Exit"] -> w272
      tunnel: [_ _ TRUE] -> w271
      tunnel: w270 -> [w277 w290 _]
      tunnel: w269 -> [w280 w288 w354]
      tunnel: [w280 w289 w354] -> w268
      tunnel: w267 -> [_ w286 _]
      tunnel: [-1 w287 _] -> w266
      tunnel: [w276 w284 _] -> w265
      tunnel: w264 -> [_ w285 w353]
      tunnel: [w274 w282 w351] -> w263
      tunnel: w262 -> [_ w283 w351]
      frame "Initialize" {
        w275 = FALSE  # your data
        n107 = call <userlib>:"CSM - Module Exit Event.vi"("Name (\"\" to Use UUID) In"=w277) -> ("CSM Exit Event"=w278:refnum<user-event>)  [unwired: 8 in, 2 out]
        n108 = register-events(w278) -> (reference out=w276:refnum<event-registration>)  [unwired: 2 in, 1 out]
        n109 = Bundle("your data"=w275) -> (w274:cluster{"your data":bool})  [unwired: 1 in]
      }
      frame "Idle", Default {
        n110 = event shown="[7] \"停止\": 值改变" {
          selector: w285 -> [_ _ _ _ _ _ _ _]
          dyn-events: [_ _ _ _ _ _ _ _] -> w284
          timeout: w286 -> [_ _ _ _ _ _ _ _]
          tunnel: [_ w298 enum16{"Idle", "Initialize", "Exit"}."Exit" _ _ _ _ _] -> w291
          tunnel: w290 -> [w293 _ _ _ _ _ _ _]
          tunnel: w288 -> [w296 w301 w313 w316 w324 w331 w338 w348]
          tunnel: [w294 w300 w313 w317 w325 w332 w339 w349] -> w289
          tunnel: [-1 _ _ _ _ _ _ _] -> w287
          tunnel: w283 -> [w292 w304 w311 w321 w328 w335 w342 w350]
          tunnel: [w292 w304 w311 w321 w328 w335 w342 w350] -> w282
          event Timeout {
            n111 = event-data() -> ()  [unwired: 1 in, 3 out]
            n112 = call-poly <userlib>:"CSM - Filter JKISM String Queue.vi"("States In"=w296) -> ("States Out"=w295:string)  [unwired: 14 in]
            n113 = call <userlib>:"CSM - Forward UI Operations to CSM.vi"("Name (\"\" to Use UUID)"=w293, "State(s) In (\"\")"=w295) -> ("States Out"=w294:string)  [unwired: 8 in, 1 out]
          }
          event Panel Close? {
            # "Wait 50ms to prevent flood of events"
            n114 = event-data() -> ()  [unwired: 1 in, 3 out]
            n115 = Two Button Dialog(message="确定关闭程序？" ("消息")) -> (T button?=w303:bool)  [unwired: 2 in]
            n116 = case shown="True" w303 {
              tunnel: w301 -> [w306 w309]
              tunnel: [w306 w308] -> w300
              tunnel: [enum16{"Idle", "Initialize", "Exit"}."Idle" enum16{"Idle", "Initialize", "Exit"}."Exit"] -> w298
              frame False {
              }
              frame True {
                n117 = call <userlib>:"CSM - Forward UI Operations to CSM.vi"("Name (\"\" to Use UUID)"=w309, "State(s) In (\"\")"="Macro: Exit" ("State")) -> ("States Out"=w308:string)  [unwired: 8 in, 1 out]
              }
            }
            n118 = event-data("Discard?"=TRUE) -> ()  [unwired: 1 in, 1 out]
          }
          event User Event {
            n119 = event-data() -> ()  [unwired: 1 in, 1 out]
          }
          event "压力采集开关": Value Change {
            n120 = event-data() -> ()  [unwired: 1 in, 1 out]
            n121 = Select(t="Macro: Start" ("State(s) in Front (\"\")"), s="压力采集开关", f="Macro: Stop" ("State(s) in Front (\"\")")) -> (s? t:f=w315:string)
            n122 = local write "压力采集-错误输出"(errorcluster {"status"=FALSE, "code"=0, "source"=""} ("压力采集-错误输出")) -> ()
            n123 = call <vilib>:"Add State(s) to Queue__JKI_lib_State_Machine.vi"("State(s) in Front (\"\")"=w315, "State(s) in (\"\")"=w316) -> ("States Out"=w317:string)  [unwired: 13 in]
          }
          event "Interval(s)": Value Change {
            n124 = event-data() -> ()  [unwired: 1 in, 1 out]
            n125 = call "Convert Data To API String Arguments.vim"("Data"="Interval(s)") -> ("API String"=w326:string)  [unwired: 7 in, 1 out]
            n126 = call <vilib>:"Build State String with Arguments__JKI_lib_State_Machine.vi"("Arguments (\"\")"=w326, "State"="API: Sample Interval" ("State(s) in Front (\"\")")) -> ("State with Arguments"=w323:string)  [unwired: 4 in]
            n127 = call <vilib>:"Add State(s) to Queue__JKI_lib_State_Machine.vi"("State(s) in Front (\"\")"=w323, "State(s) in (\"\")"=w324) -> ("States Out"=w325:string)  [unwired: 13 in]
          }
          event "压力串口": Value Change {
            n128 = event-data() -> ()  [unwired: 1 in, 1 out]
            n129 = call "Convert Data To API String Arguments.vim"("Data"="压力串口") -> ("API String"=w333:string)  [unwired: 7 in, 1 out]
            n130 = call <vilib>:"Build State String with Arguments__JKI_lib_State_Machine.vi"("Arguments (\"\")"=w333, "State"="API: USB Port " ("State(s) in Front (\"\")")) -> ("State with Arguments"=w330:string)  [unwired: 4 in]
            n131 = call <vilib>:"Add State(s) to Queue__JKI_lib_State_Machine.vi"("State(s) in Front (\"\")"=w330, "State(s) in (\"\")"=w331) -> ("States Out"=w332:string)  [unwired: 13 in]
          }
          event "压力设备选择": Value Change {
            n132 = event-data() -> ()  [unwired: 1 in, 1 out]
            n133 = call "Convert Data To API String Arguments.vim"("Data"="压力设备选择") -> ("API String"=w340:string)  [unwired: 7 in, 1 out]
            n134 = call <vilib>:"Build State String with Arguments__JKI_lib_State_Machine.vi"("Arguments (\"\")"=w340, "State"="API: Dev Choose" ("State(s) in Front (\"\")")) -> ("State with Arguments"=w337:string)  [unwired: 4 in]
            n135 = call <vilib>:"Add State(s) to Queue__JKI_lib_State_Machine.vi"("State(s) in Front (\"\")"=w337, "State(s) in (\"\")"=w338) -> ("States Out"=w339:string)  [unwired: 13 in]
          }
          event "停止": Value Change {
            n136 = event-data() -> ()  [unwired: 1 in, 1 out]
            n137 = Two Button Dialog(message="确定停止程序？" ("消息")) -> (T button?=w345:bool)  [unwired: 2 in]
            n138 = Select(t="Macro: Exit" ("State(s) in Front (\"\")"), s=w345, f="") -> (s? t:f=w343:string)
            n139 = call <vilib>:"Add State(s) to Queue__JKI_lib_State_Machine.vi"("State(s) in Front (\"\")"=w343, "State(s) in (\"\")"=w348) -> ("States Out"=w349:string)  [unwired: 13 in]
          }
        }
      }
      frame "Exit" {
        n140 = Unregister For Events(event registration refnum=w353) -> (error out=w352:errorcluster)  [unwired: 1 in]
        n141 = call <vilib>:"Clear Errors.vi"("error in (no error)"=w352) -> ()  [unwired: 5 in, 2 out]
      }
    }
  }
  n142 = flat-sequence {
    tunnel: "子程序？" -> [w357]
    tunnel: "CSM Name" -> [w359]
    frame #0 {
      n143 = Concatenate Strings("Acquisition - " ("Name(\"\" to use uuid)"), w359) -> (w360:string)
      n144 = call "Acquisition.vi"("CSM Name"=w360) -> ()  [unwired: 11 in]
      n145 = Concatenate Strings("Logging - " ("Name(\"\" to use uuid)"), w359) -> (w358:string)
      n146 = case shown="False" w357 {
        tunnel: w358 -> [w363 _]
        frame False {
          n147 = call "Logging.vi"("CSM Name"=w363) -> ()  [unwired: 11 in]
        }
        frame True {
        }
      }
    }
  }
  n148 = call <userlib>:"CSM - Sync Configuration Variables to File.vi"("All Temp Variable to Default Ini(F)"=TRUE, "error in (no error)"=w4) -> ()  [unwired: 7 in, 1 out]
